vi "Get_MultiVar_BulkMode_Value.vi"(8 "error in (no error)":errorcluster, 10 "varName":string, 11 "muExpr in":refnum<class "mupExpr.lvclass">) -> (0 "error out":errorcluster, 2 "Values":dbl[](array[numeric]), 3 "muExpr out":refnum<class "mupExpr.lvclass">)   [LabVIEW 2015, in "mupExpr.lvclass"]
doc: "Lookup variable's bulk mode values by name."
uses:
  mupExpr.lvclass
  mupExpr.lvclass/mupExpr.ctl
  <vilib>/Utility/error.llb/Error Cluster From Error Code.vi
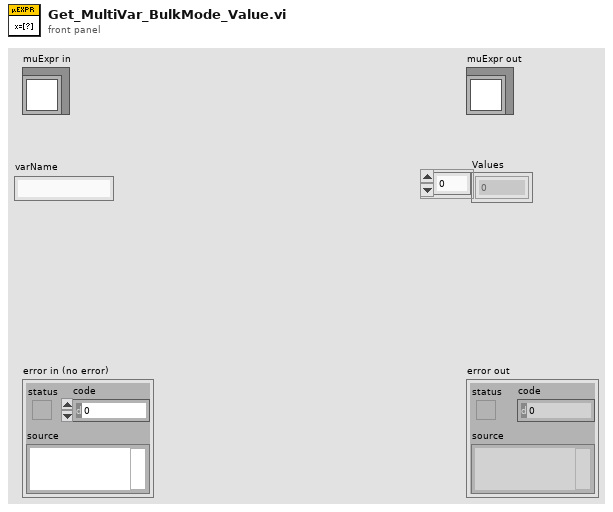
[diagram p1: front panel]
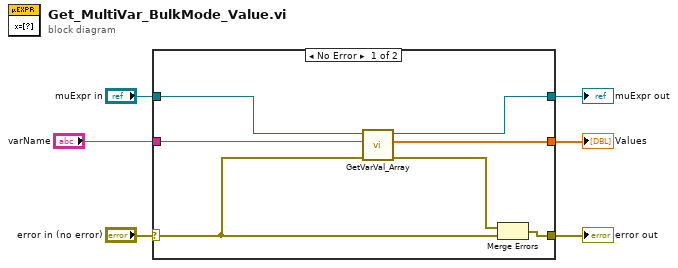
[diagram p0: block diagram]
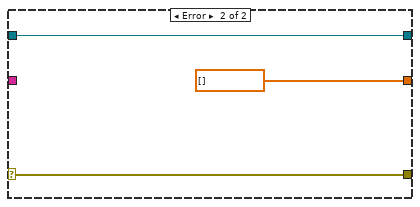
[diagram p2: hidden frame]
diagram:
  n1 = case shown="No Error" "error in (no error)" {
    selector: "error in (no error)" -> [w9 w16]
    tunnel: [w11 w16] -> w5
    tunnel: [w8 w15] -> w3
    tunnel: "muExpr in" -> [w7 w15]
    tunnel: [w13 dbl[] [] ("pd")] -> w2
    tunnel: "varName" -> [w10 _]
    frame No Error {
      n2 = call "GetVarVal_Array.vi"("error in (no error)"=w9, "varName"=w10, "muExpr in"=w7) -> ("error out"=w12:errorcluster, "varValue"=w13:dbl[], "muExpr out"=w8:refnum<class "mupExpr.lvclass">)  [unwired: 6 in]
      n3 = Merge Errors(w12, w9) -> (w11:errorcluster)
    }
    frame Error {
    }
  }
  "error out" <- w5
  "muExpr out" <- w3
  "Values" <- w2
